vi "Global Variable.vi"() -> ()   [LabVIEW 2020]
doc: "111234"
panel:
  in  "Global Thing":string caption="Caption"
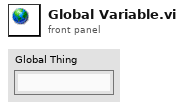
[diagram p1: front panel]
diagram:
